vi "Silver--constant.vi"() -> (1 "Silver":u32(colorbox))   [LabVIEW 2018, in "Band Colors.lvlib"]
doc: "Provides the RGB color value for silver.\n\nThe VI converts the RGB components (192, 192, 192) into a LabVIEW color value and returns it through <b>Silver</b>."
uses:
  Band Colors.lvlib
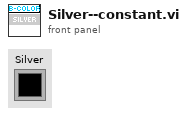
[diagram p1: front panel]
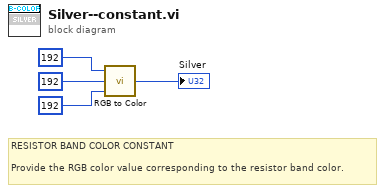
[diagram p0: block diagram]
diagram:
  # "RESISTOR BAND COLOR CONSTANT\n\nProvide the RGB color value corresponding to the resistor band color."
  n1 = call <vilib>:"RGB to Color.vi"("B"=u8 192, "G"=u8 192, "R"=u8 192) -> ("Color"=→"Silver":u32)
